vi "GetVIText.vi"(8 "error in (no error)":errorcluster, 10 "Control Name (Blank = All controls in VI)":string, 11 "VI":refnum<vi>) -> (0 "error out":errorcluster, 1 "Font Name":string, 2 "Control Text":string[](array[string]), 3 "Control Keys":string[](array[string]))   [LabVIEW 2017]
uses:
  <vilib>/Utility/traverseref.llb/TRef TravTarget.ctl
  <vilib>/Utility/traverseref.llb/VI Scripting - Traverse.lvlib
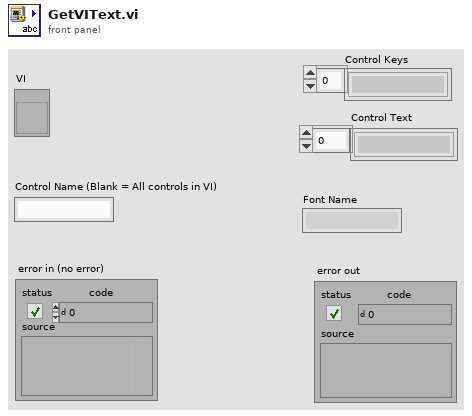
[diagram p1: front panel]
types:
  T1 = typedef "TRef TravTarget.ctl" = enum16{"FP", "BD", "Other"}
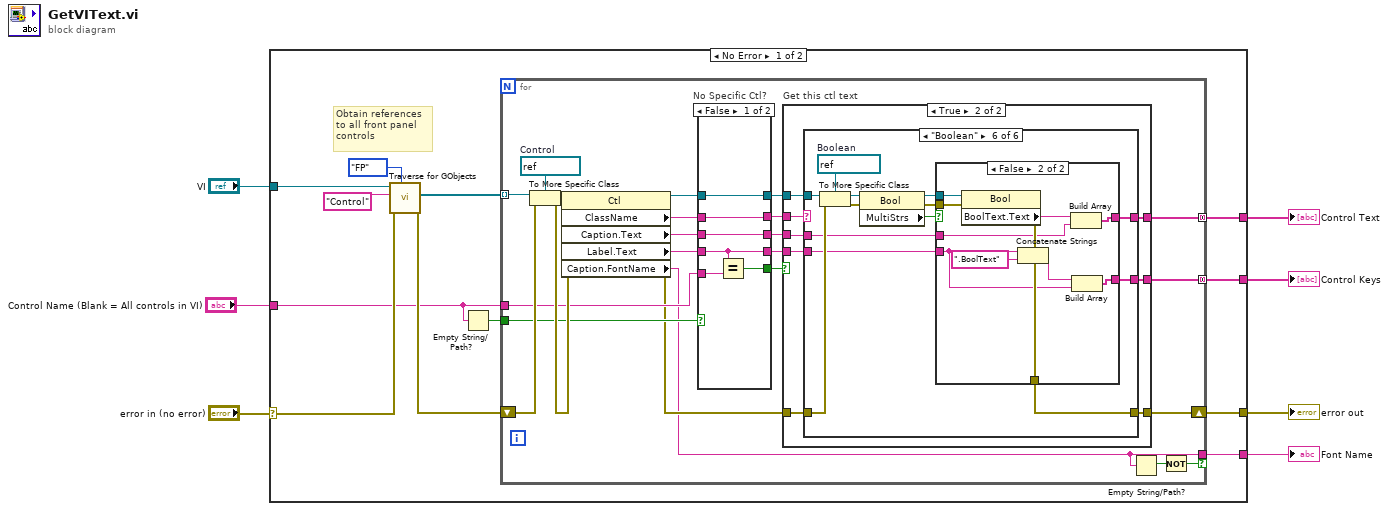
[diagram p0: block diagram]
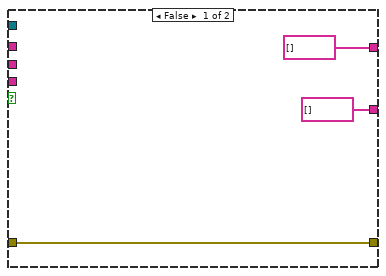
[diagram p2: hidden frame]
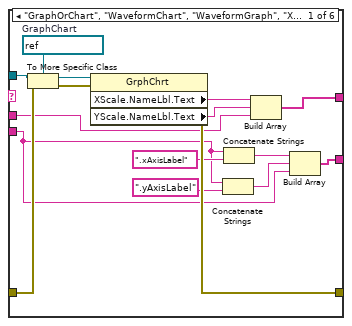
[diagram p3: hidden frame]
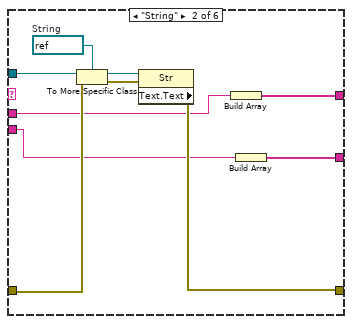
[diagram p4: hidden frame]
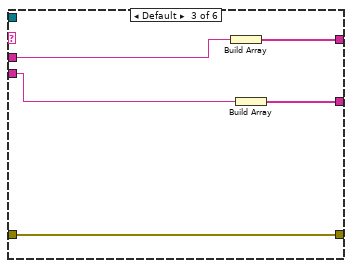
[diagram p5: hidden frame]
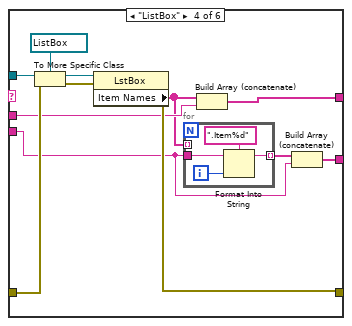
[diagram p6: hidden frame]
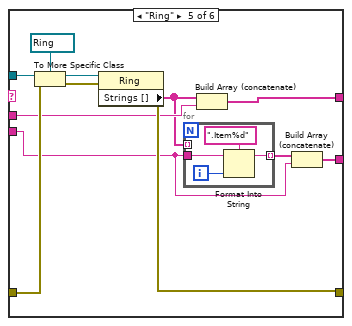
[diagram p7: hidden frame]
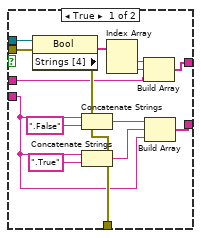
[diagram p8: hidden frame]
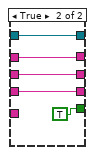
[diagram p9: hidden frame]
diagram:
  n1 = case shown="No Error" "error in (no error)" {
    selector: "error in (no error)" -> [w15 w165]
    tunnel: "VI" -> [w17 _]
    tunnel: "Control Name (Blank = All controls in VI)" -> [w11 _]
    tunnel: [w13 w165] -> w4
    tunnel: [w10 _] -> w3
    tunnel: [w9 _] -> w2
    tunnel: [w8 _] -> w1
    frame No Error {
      # "Obtain references to all front panel controls"
      n2 = call <vilib>:"Traverse for GObjects.vi"("Traverse Target"=TRef_TravTarget."FP", "error in (no error)"=w15, "Class Name"="Control", "VI Refnum"=w17) -> ("error out"=w14:errorcluster, "References"=w16:refnum<vi>[])  [unwired: 4 in, 2 out]
      n3 = Empty String/Path?(string/path=w11) -> (empty?=w12:bool)
      n4 = for {
        tunnel: w16 -> [w42] mode=indexing
        shift-right: [w31] -> w13
        shift-left: w14 -> [w39]
        tunnel: w11 -> [w37]
        tunnel: w12 -> [w35]
        tunnel: [w24] -> w10 mode=concatenating
        tunnel: [w23] -> w9 mode=concatenating
        tunnel: [w22] -> w8 if=w20
        w40 = refnum<vi> refnum  # Control
        n5 = To More Specific Class(target class=w40, reference=w42, error in=w39) -> (specific class reference=w41:refnum<vi>, error out=w38:errorcluster)
        n6 = property class="Ctl"(reference=w41, error in=w38) -> (reference out=w25:refnum<vi>, error out=w32:errorcluster, "ClassName"=w34:string, "Caption.Text"=w33:string, "Label.Text"=w36:string, "Caption.FontName"=w22:string)
        n7 = case "No Specific Ctl?" shown="False" w35 {
          tunnel: w37 -> [w159 _]
          tunnel: w36 -> [w157 w161]
          tunnel: w34 -> [w155 w164]
          tunnel: w33 -> [w156 w162]
          tunnel: [w158 TRUE] -> w30
          tunnel: [w155 w164] -> w27
          tunnel: [w156 w162] -> w29
          tunnel: [w157 w161] -> w28
          tunnel: [w154 w160] -> w26
          tunnel: w25 -> [w154 w160]
          frame False {
            n8 = Equal?(x=w157, y=w159) -> (x = y?=w158:bool)
          }
          frame True {
          }
        }
        n9 = case "Get this ctl text" shown="True" w30 {
          tunnel: w32 -> [w45 w51]
          tunnel: [w45 w50] -> w31
          tunnel: w29 -> [_ w48]
          tunnel: w28 -> [_ w49]
          tunnel: w27 -> [_ w53]
          tunnel: w26 -> [_ w52]
          tunnel: [string[] [] w47] -> w24
          tunnel: [string[] [] w46] -> w23
          frame False {
          }
          frame True {
            n10 = case shown="\"Boolean\"" w53 {
              tunnel: w52 -> [w66 w76 _ w93 w109 w128]
              tunnel: w51 -> [w65 w75 w84 w92 w108 w127]
              tunnel: [w64 w74 w84 w91 w107 w126] -> w50
              tunnel: [w63 w73 w83 w90 w106 w125] -> w47
              tunnel: w49 -> [w55 w71 w81 w86 w102 w123]
              tunnel: w48 -> [w62 w72 w82 w89 w105 w124]
              tunnel: [w54 w70 w80 w85 w101 w122] -> w46
              frame "GraphOrChart", "WaveformChart", "WaveformGraph", "XYGraph" {
                w68 = refnum<vi> refnum  # GraphChart
                n11 = To More Specific Class(target class=w68, reference=w66, error in=w65) -> (specific class reference=w69:refnum<vi>, error out=w67:errorcluster)
                n12 = property class="GrphChrt"(reference=w69, error in=w67) -> (error out=w64:errorcluster, "XScale.NameLbl.Text"=w59:string, "YScale.NameLbl.Text"=w58:string)  [unwired: 1 out]
                n13 = Concatenate Strings(w55, ".yAxisLabel" ("string")) -> (w56:string)
                n14 = Concatenate Strings(w55, ".xAxisLabel" ("string")) -> (w57:string)
                n15 = Build Array(w59, w58, w62) -> (w63:string[])
                n16 = Build Array(w57, w56, w55) -> (w54:string[])
              }
              frame "String" {
                w79 = refnum<vi> refnum  # String
                n17 = To More Specific Class(target class=w79, reference=w76, error in=w75) -> (specific class reference=w78:refnum<vi>, error out=w77:errorcluster)
                n18 = property class="Str" props=["Text", "Text"](reference=w78, error in=w77) -> (error out=w74:errorcluster)  [unwired: 2 out]
                n19 = Build Array(w72) -> (w73:string[])
                n20 = Build Array(w71) -> (w70:string[])
              }
              frame Default {
                n21 = Build Array(w82) -> (w83:string[])
                n22 = Build Array(w81) -> (w80:string[])
              }
              frame "ListBox" {
                n23 = To More Specific Class(target class=refnum<vi> refnum ("reference out"), reference=w93, error in=w92) -> (specific class reference=w96:refnum<vi>, error out=w95:errorcluster)
                n24 = property class="LstBox"(reference=w96, error in=w95) -> (error out=w91:errorcluster, "Item Names"=w88:string[])  [unwired: 1 out]
                n25 = for {
                  tunnel: w86 -> [w100]
                  tunnel: w88 -> [_] mode=indexing
                  tunnel: [w97] -> w87 mode=indexing
                  i -> [w98]
                  n26 = Format Into String(format string=".Item%d", initial string=w100, w98) -> (resulting string=w97:string)  [unwired: 1 in, 1 out]
                }
                n27 = Build Array (concatenate)(w88, w89) -> (w90:string[])
                n28 = Build Array (concatenate)(w87, w86) -> (w85:string[])
              }
              frame "Ring" {
                n29 = To More Specific Class(target class=refnum<vi> refnum ("reference out"), reference=w109, error in=w108) -> (specific class reference=w112:refnum<vi>, error out=w111:errorcluster)
                n30 = property class="Ring"(reference=w112, error in=w111) -> (error out=w107:errorcluster, "Strings []"=w104:string[])  [unwired: 1 out]
                n31 = for {
                  tunnel: w102 -> [w116]
                  tunnel: w104 -> [_] mode=indexing
                  tunnel: [w113] -> w103 mode=indexing
                  i -> [w114]
                  n32 = Format Into String(format string=".Item%d", initial string=w116, w114) -> (resulting string=w113:string)  [unwired: 1 in, 1 out]
                }
                n33 = Build Array (concatenate)(w104, w105) -> (w106:string[])
                n34 = Build Array (concatenate)(w103, w102) -> (w101:string[])
              }
              frame "Boolean" {
                w129 = refnum<vi> refnum  # Boolean
                n35 = To More Specific Class(target class=w129, reference=w128, error in=w127) -> (specific class reference=w121:refnum<vi>, error out=w119:errorcluster)
                n36 = property class="Bool"(reference=w121, error in=w119) -> (reference out=w120:refnum<vi>, error out=w118:errorcluster, "MultiStrs"=w117:bool)
                n37 = case shown="False" w117 {
                  tunnel: [w143 w148] -> w126
                  tunnel: [w141 w152] -> w125
                  tunnel: w124 -> [w130 w144]
                  tunnel: w123 -> [w136 w145]
                  tunnel: [w135 w151] -> w122
                  tunnel: w120 -> [w134 w150]
                  tunnel: w118 -> [w133 w149]
                  frame True {
                    n38 = property class="Bool"(reference=w134, error in=w133) -> (error out=w143:errorcluster, "Strings [4]"=w142:string[])  [unwired: 1 out]
                    n39 = Concatenate Strings(w136, ".False" ("string")) -> (w139:string)
                    n40 = Concatenate Strings(w136, ".True" ("string")) -> (w137:string)
                    n41 = Index Array(array=w142) -> (element #1=w132:string, element #2=w131:string)  [unwired: 2 in]
                    n42 = Build Array(w132, w131, w130) -> (w141:string[])
                    n43 = Build Array(w139, w137, w136) -> (w135:string[])
                  }
                  frame False {
                    n44 = property class="Bool"(reference=w150, error in=w149) -> (error out=w148:errorcluster, "BoolText.Text"=w153:string)  [unwired: 1 out]
                    n45 = Concatenate Strings(w145, ".BoolText" ("string")) -> (w147:string)
                    n46 = Build Array(w153, w144) -> (w152:string[])
                    n47 = Build Array(w147, w145) -> (w151:string[])
                  }
                }
              }
            }
          }
        }
        n48 = Empty String/Path?(string/path=w22) -> (empty?=w21:bool)
        n49 = Not(x=w21) -> (.not. x?=w20:bool)
      }
    }
    frame Error {
    }
  }
  "Control Text" <- w3
  "error out" <- w4
  "Control Keys" <- w2
  "Font Name" <- w1
